vi "ASM A_PATH formation.vi"(8 "error in (no error)":errorcluster caption="エラー入力（エラーなし）", 11 "F_name":path=path "D:/MCBJ data/Micro RNA Data/let7f W22/00 Good Signal") -> (0 "error out":errorcluster, 1 "AR Table Path":path, 2 "info Cluster":T2, 3 "SRBJT Path":T3, 4 "Path_Name":T1)   [LabVIEW 2018]
panel:
  out "after substring 3":string
  out "name 2":string
  out "after substring 2":string
  out "concatenated string 3":string
  out "after substring":string
  out "concatenated string 2":string
  out "BSX Path":path
  out "PSX Path":path
  out "B_Table_name":string
  out "R_Table_name":string
  out "S_Table_name":string
  out "Folder_name":string
  out "File_headername":string
  out "concatenated string":string
  out "name":string
  out "日付/時間文字列":string
  out "Filename":string
  out "JPEG Path":path
  out "A TDMS Path":path
  out "B Table Path":path
  out "D con":string
  out "A New folder":string
  out "AN time":string
  out "Ainfo":string
  out "F ex Info":T4
  out "R Table Path":path
  out "S Table Path":path
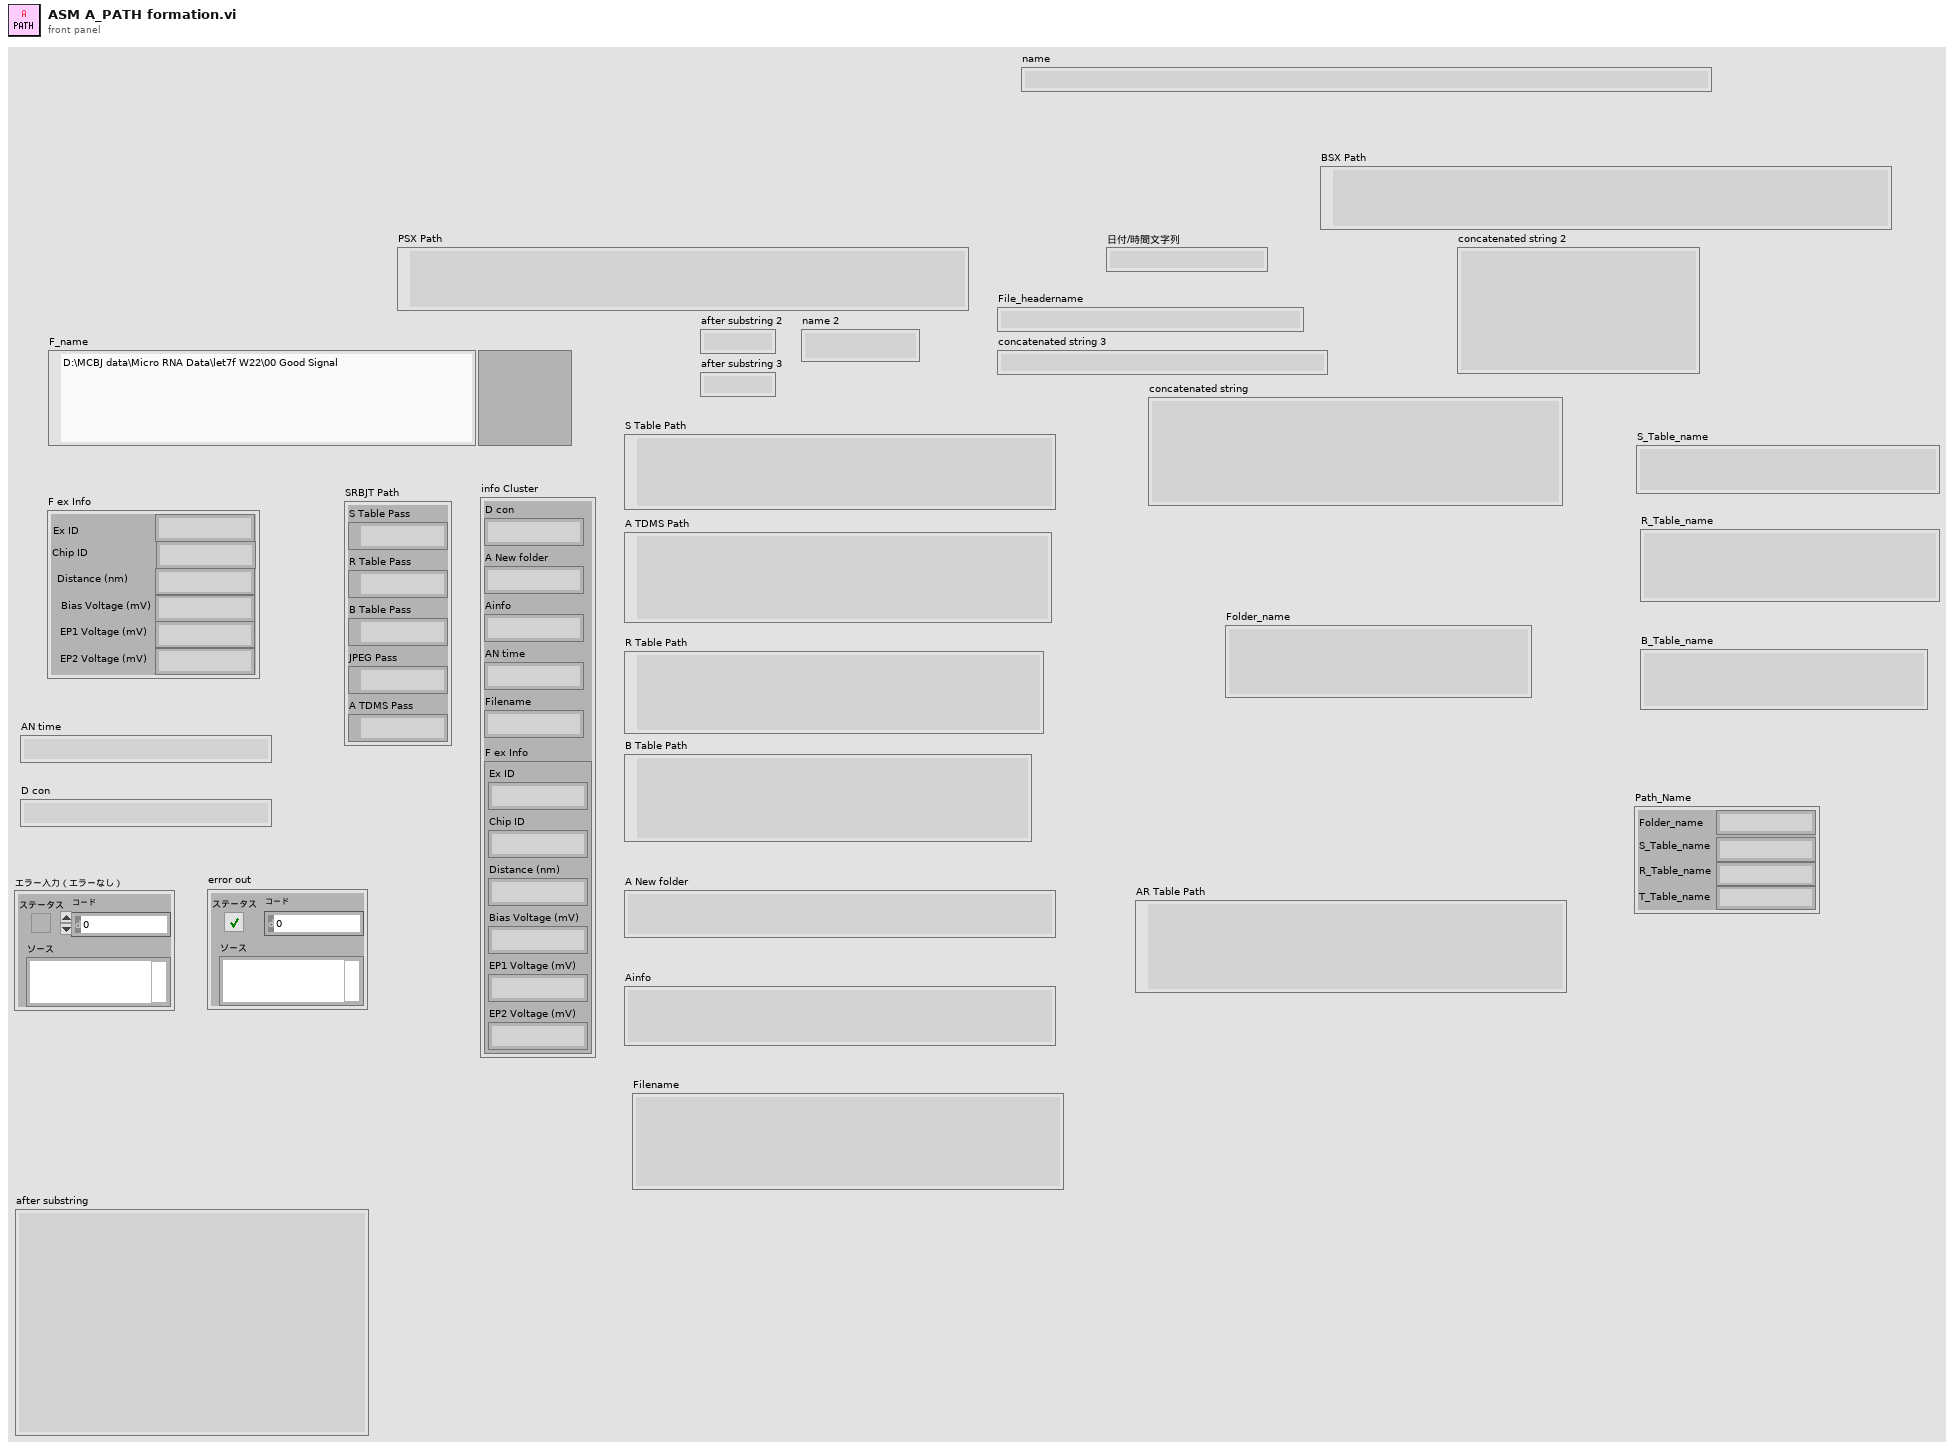
[diagram p1: front panel]
types:
  T1 = cluster{"Folder_name":string, "S_Table_name":string, "R_Table_name":string, "T_Table_name":string}
  T2 = cluster{"D con":string, "A New folder":string, "Ainfo":string, "AN time":string, "Filename":string, "F ex Info":cluster{"Ex ID":string, "Chip ID":string, "Distance (nm)":string, "Bias Voltage (mV)":string, "EP1 Voltage (mV)":string, "EP2 Voltage (mV)":string}}
  T3 = cluster{"S Table Pass":path, "R Table Pass":path, "B Table Pass":path, "JPEG Pass":path, "A TDMS Pass":path}
  T4 = cluster{"Ex ID":string, "Chip ID":string, "Distance (nm)":string, "Bias Voltage (mV)":string, "EP1 Voltage (mV)":string, "EP2 Voltage (mV)":string}
  T5 = cluster{"文字列":string, string, string, "date/time string":string, "name":string, "F ex Info":cluster{"Ex ID":string, "Chip ID":string, "Distance (nm)":string, "Bias Voltage (mV)":string, "EP1 Voltage (mV)":string, "EP2 Voltage (mV)":string}}
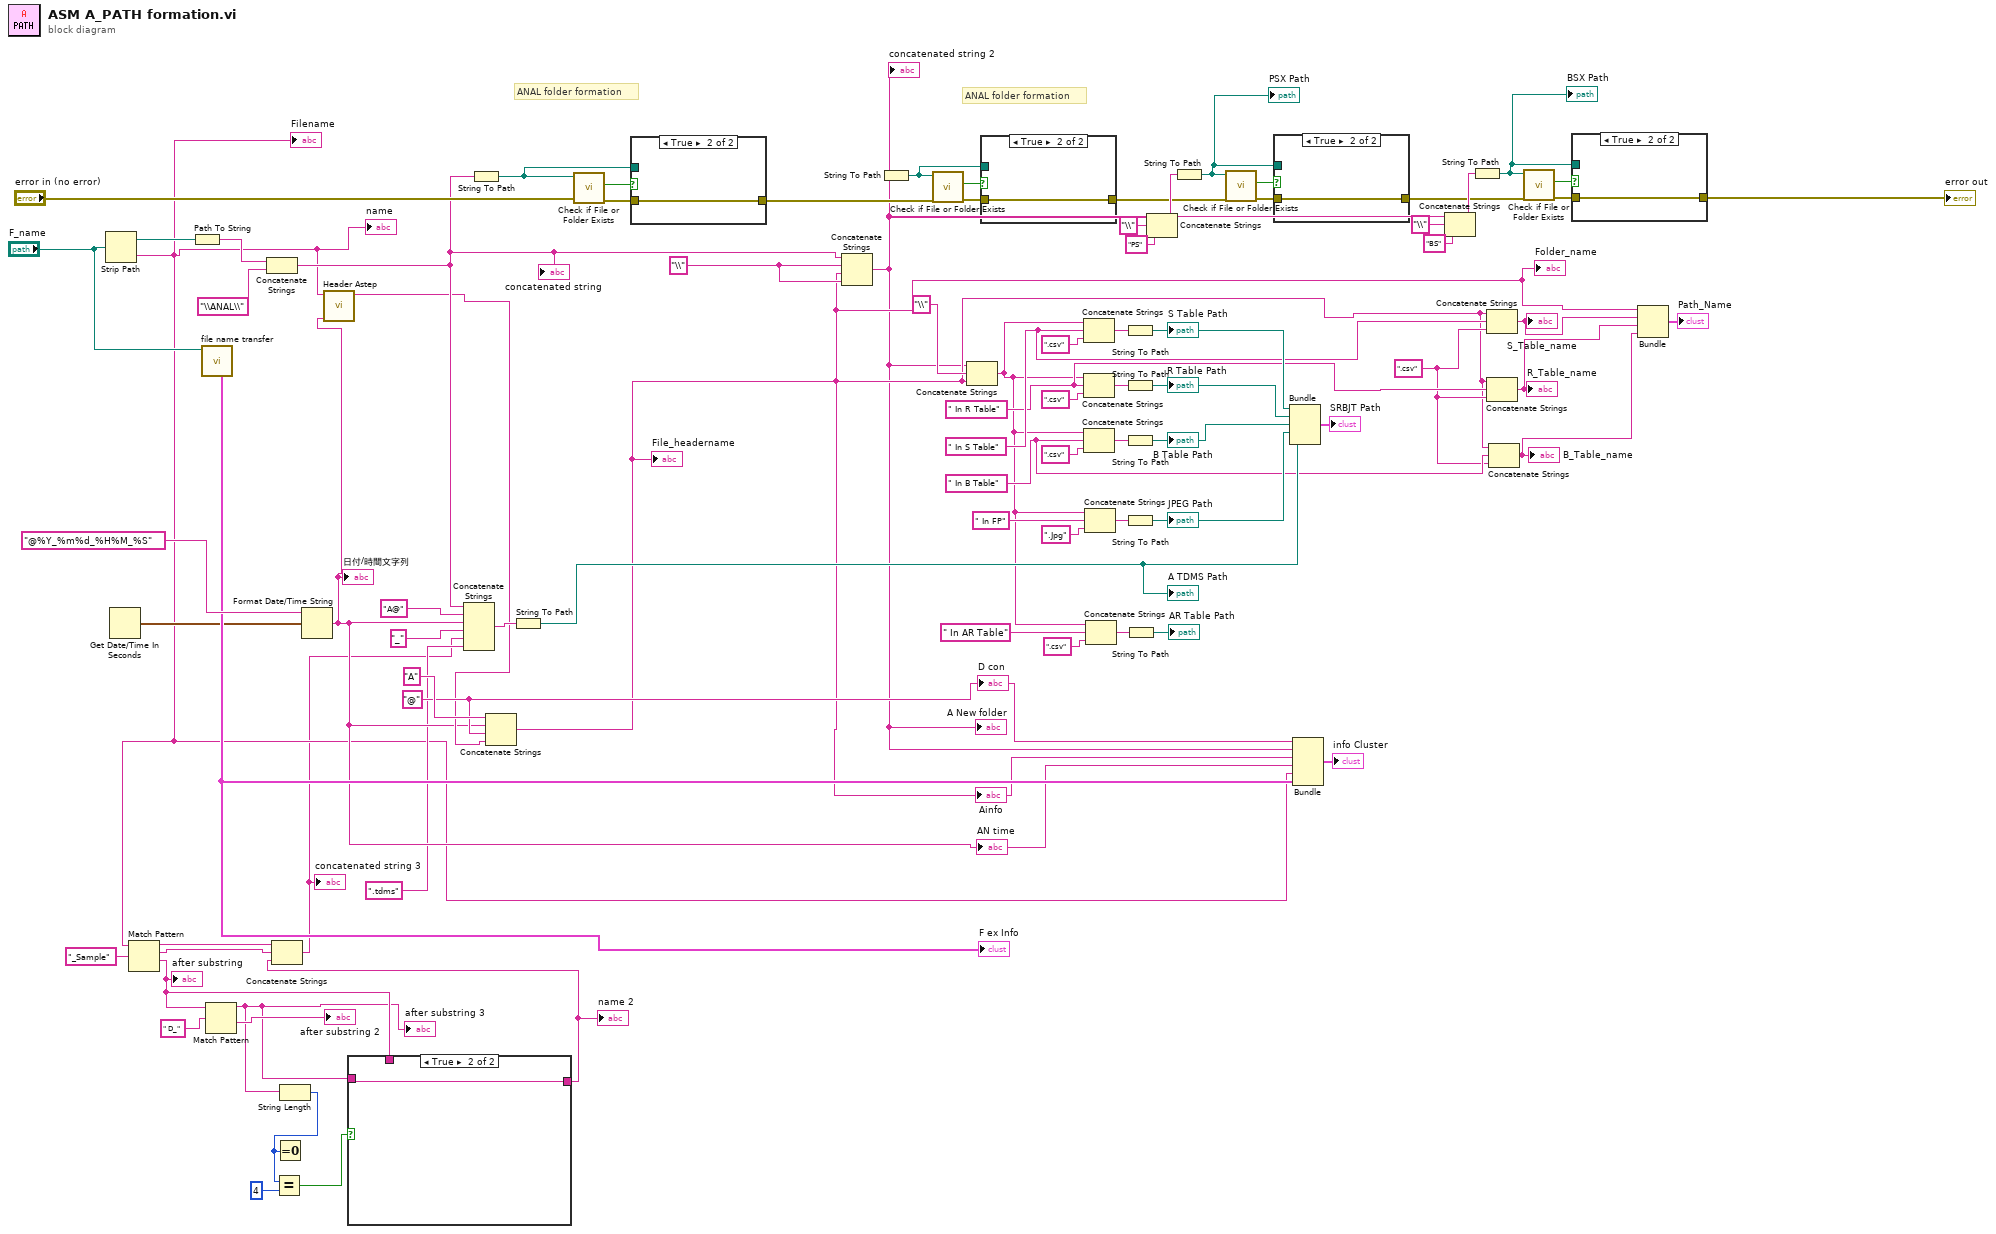
[diagram p0: block diagram]
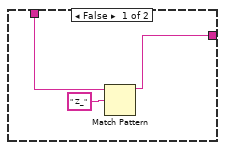
[diagram p2: hidden frame]
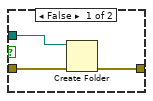
[diagram p3: hidden frame]
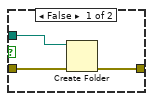
[diagram p4: hidden frame]
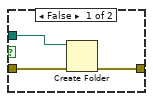
[diagram p5: hidden frame]
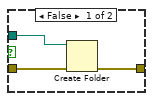
[diagram p6: hidden frame]
diagram:
  w37 = ".csv" ("format (%.3f)")
  w50 = "@" ("文字列")
  w60 = "\\" ("文字列")
  w38 = " In B Table" ("文字列")
  w39 = " In R Table" ("文字列")
  w40 = " In S Table" ("文字列")
  # "ANAL folder formation"
  # "ANAL folder formation"
  n1 = Strip Path(path="F_name") -> (stripped path=w83:path, name=w9:string)
  "Filename" <- w9
  "name" <- w9
  n2 = Get Date/Time In Seconds() -> (seconds since 1Jan1904=w42:timestamp)
  n3 = Match Pattern(string=w9, regular expression="_Sample") -> (before substring=w11:string, match substring=w10:string, after substring=w5:string)  [unwired: 1 in, 1 out]
  "after substring" <- w5
  n4 = Path To String(path=w83) -> (string=w49:string)
  n5 = call "file name transfer.vi"("パス"="F_name") -> ("F ex Info"=w51:T4)  [unwired: 6 in, 4 out]
  "F ex Info" <- w51
  n6 = Match Pattern(string=w5, regular expression=" D_") -> (before substring=w4:string, after substring=→"after substring 2":string)  [unwired: 1 in, 2 out]
  "after substring 3" <- w4
  n7 = Concatenate Strings(w49, "\\ANAL\\" ("文字列")) -> (w61:string)
  "concatenated string" <- w61
  n8 = String Length(string=w4) -> (length=w3:i32)
  n9 = Equal?(x=w3, y=4) -> (x = y?=w1:bool)
  n10 = Equal To 0?(x=w3) -> ()  [unwired: 1 out]
  n11 = Format Date/Time String(time format string (%c)="@%Y_%m%d_%H%M_%S" ("時間形式文字列（%c）"), seconds (now)=w42) -> (date/time string=w41:string)  [unwired: 1 in]
  "AN time" <- w41
  "日付/時間文字列" <- w41
  n12 = call "Header Astep.vi"("日付/時間文字列"=w41, "文字列"=w9) -> ("Header for Astep"=w47:string)  [unwired: 9 in]
  n13 = case shown="True" w1 {
    tunnel: [w86 w89] -> w6
    tunnel: w4 -> [_ w89]
    tunnel: w5 -> [w87 _]
    frame False {
      n14 = Match Pattern(string=w87, regular expression=" Z_") -> (before substring=w86:string)  [unwired: 1 in, 3 out]
    }
    frame True {
    }
  }
  "name 2" <- w6
  n15 = Concatenate Strings(w11, w10, w6) -> (w8:string)
  "concatenated string 3" <- w8
  n16 = Concatenate Strings(w61, "A@" ("文字列"), w41, "_" ("文字列"), w8, ".tdms" ("string")) -> (w71:string)
  n17 = String To Path(string=w61) -> (path=w82:path)
  n18 = Concatenate Strings("A" ("文字列"), w41, w50, w47) -> (w36:string)
  "Ainfo" <- w36
  "File_headername" <- w36
  "Folder_name" <- w36
  n19 = String To Path(string=w71) -> (path=w57:path)
  "A TDMS Path" <- w57
  n20 = call <vilib>:"Check if File or Folder Exists.vi"("error in (no error)"="error in (no error)", "path"=w82) -> ("error out"=w80:errorcluster, "file or folder exists?"=w81:bool)  [unwired: 7 in, 1 out]
  n21 = case shown="True" w81 {
    tunnel: w82 -> [w92 _]
    tunnel: w80 -> [w91 w93]
    tunnel: [w90 w93] -> w63
    frame False {
      n22 = Create Folder(path (use dialog)=w92, error in=w91) -> (error out=w90:errorcluster)  [unwired: 1 in, 2 out]
    }
    frame True {
    }
  }
  n23 = Concatenate Strings(w61, w60, w36, w60) -> (w15:string)
  "A New folder" <- w15
  "concatenated string 2" <- w15
  n24 = String To Path(string=w15) -> (path=w66:path)
  n25 = call <vilib>:"Check if File or Folder Exists.vi"("error in (no error)"=w63, "path"=w66) -> ("error out"=w64:errorcluster, "file or folder exists?"=w65:bool)  [unwired: 7 in, 1 out]
  n26 = Concatenate Strings(w15, "\\" ("文字列"), w36) -> (w16:string)
  n27 = case shown="True" w65 {
    tunnel: w66 -> [w96 _]
    tunnel: w64 -> [w95 w97]
    tunnel: [w94 w97] -> w25
    frame False {
      n28 = Create Folder(path (use dialog)=w96, error in=w95) -> (error out=w94:errorcluster)  [unwired: 1 in, 2 out]
    }
    frame True {
    }
  }
  n29 = Concatenate Strings(w16, w40, ".csv" ("format (%.3f)")) -> (w75:string)
  n30 = Concatenate Strings(w16, w39, ".csv" ("format (%.3f)")) -> (w76:string)
  n31 = Concatenate Strings(w16, w38, ".csv" ("format (%.3f)")) -> (w73:string)
  n32 = Concatenate Strings(w16, " In FP" ("文字列"), ".Jpg" ("format (%.3f)")) -> (w68:string)
  n33 = Concatenate Strings(w16, " In AR Table" ("文字列"), ".csv" ("format (%.3f)")) -> (w44:string)
  n34 = String To Path(string=w75) -> (path=w53:path)
  "S Table Path" <- w53
  n35 = String To Path(string=w76) -> (path=w54:path)
  "R Table Path" <- w54
  n36 = String To Path(string=w73) -> (path=w55:path)
  "B Table Path" <- w55
  n37 = String To Path(string=w68) -> (path=w56:path)
  "JPEG Path" <- w56
  n38 = String To Path(string=w44) -> (path=→"AR Table Path":path)
  n39 = Concatenate Strings(w15, "\\" ("string"), "PS" ("string")) -> (w27:string)
  n40 = String To Path(string=w27) -> (path=w26:path)
  "PSX Path" <- w26
  n41 = call <vilib>:"Check if File or Folder Exists.vi"("error in (no error)"=w25, "path"=w26) -> ("error out"=w30:errorcluster, "file or folder exists?"=w31:bool)  [unwired: 7 in, 1 out]
  n42 = case shown="True" w31 {
    tunnel: w26 -> [w100 _]
    tunnel: w30 -> [w99 w101]
    tunnel: [w98 w101] -> w18
    frame False {
      n43 = Create Folder(path (use dialog)=w100, error in=w99) -> (error out=w98:errorcluster)  [unwired: 1 in, 2 out]
    }
    frame True {
    }
  }
  n44 = Bundle(w53, w54, w55, w56, w57) -> (→"SRBJT Path":cluster{path, path, path, path, path})  [unwired: 1 in]
  n45 = Bundle("文字列"=w50, w15, w36, "date/time string"=w41, "name"=w9, "F ex Info"=w51) -> (→"info Cluster":T5)  [unwired: 1 in]
  n46 = Concatenate Strings(w15, "\\" ("string"), "BS" ("string")) -> (w20:string)
  n47 = String To Path(string=w20) -> (path=w19:path)
  "BSX Path" <- w19
  n48 = Concatenate Strings(w36, w40, w37) -> (w35:string)
  "S_Table_name" <- w35
  n49 = Concatenate Strings(w36, w39, w37) -> (w34:string)
  "R_Table_name" <- w34
  n50 = Concatenate Strings(w36, w38, w37) -> (w33:string)
  "B_Table_name" <- w33
  n51 = call <vilib>:"Check if File or Folder Exists.vi"("error in (no error)"=w18, "path"=w19) -> ("error out"=w23:errorcluster, "file or folder exists?"=w24:bool)  [unwired: 7 in, 1 out]
  n52 = case shown="True" w24 {
    tunnel: w19 -> [w104 _]
    tunnel: w23 -> [w103 w105]
    tunnel: [w102 w105] -> w17
    frame False {
      n53 = Create Folder(path (use dialog)=w104, error in=w103) -> (error out=w102:errorcluster)  [unwired: 1 in, 2 out]
    }
    frame True {
    }
  }
  "error out" <- w17
  n54 = Bundle(w36, w35, w34, w33) -> (→"Path_Name":cluster{string, string, string, string})  [unwired: 1 in]
  "D con" <- w50
